vi "PayloadHPLP.vi"(8 "Modulation type LP":enum16{"QPSK(4QAM)", "64QAM", "16QAM", "BPSK"}(ring), 11 "Modulation type HP":enum16{"QPSK(4QAM)", "64QAM", "16QAM", "BPSK"}(ring)) -> (2 "Payload_LP":i32=720, 3 "Payload_HP":i32=720)   [LabVIEW 2022 SP3]
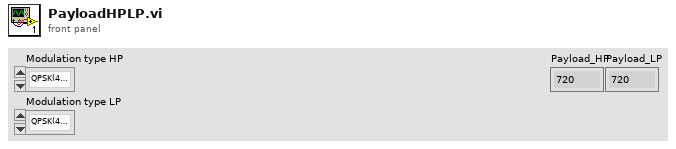
[diagram p1: front panel]
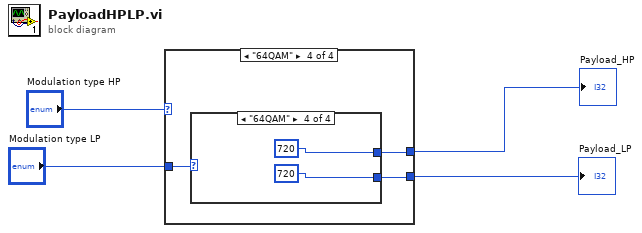
[diagram p0: block diagram]
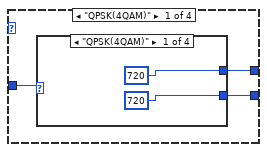
[diagram p2: hidden frame]
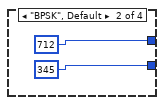
[diagram p3: hidden frame]
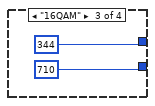
[diagram p4: hidden frame]
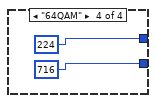
[diagram p5: hidden frame]
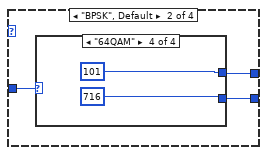
[diagram p6: hidden frame]
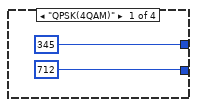
[diagram p7: hidden frame]
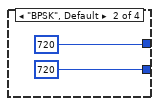
[diagram p8: hidden frame]
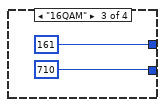
[diagram p9: hidden frame]
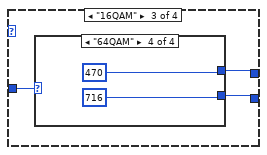
[diagram p10: hidden frame]
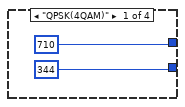
[diagram p11: hidden frame]
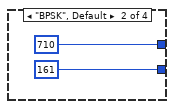
[diagram p12: hidden frame]
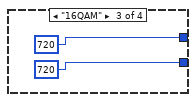
[diagram p13: hidden frame]
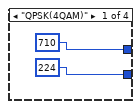
[diagram p14: hidden frame]
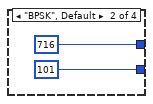
[diagram p15: hidden frame]
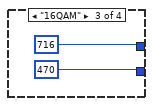
[diagram p16: hidden frame]
diagram:
  n1 = case shown="\"64QAM\"" "Modulation type HP" {
    tunnel: "Modulation type LP" -> [w7 w18 w29 w40]
    tunnel: [w6 w17 w28 w39] -> w2
    tunnel: [w5 w16 w27 w38] -> w1
    frame "QPSK(4QAM)" {
      n2 = case shown="\"QPSK(4QAM)\"" w7 {
        tunnel: [720 712 344 224] -> w6
        tunnel: [720 345 710 716] -> w5
        frame "QPSK(4QAM)" {
        }
        frame "BPSK", Default {
        }
        frame "16QAM" {
        }
        frame "64QAM" {
        }
      }
    }
    frame "BPSK", Default {
      n3 = case shown="\"64QAM\"" w18 {
        tunnel: [345 720 161 101] -> w17
        tunnel: [712 720 710 716] -> w16
        frame "QPSK(4QAM)" {
        }
        frame "BPSK", Default {
        }
        frame "16QAM" {
        }
        frame "64QAM" {
        }
      }
    }
    frame "16QAM" {
      n4 = case shown="\"64QAM\"" w29 {
        tunnel: [710 710 720 470] -> w28
        tunnel: [344 161 720 716] -> w27
        frame "QPSK(4QAM)" {
        }
        frame "BPSK", Default {
        }
        frame "16QAM" {
        }
        frame "64QAM" {
        }
      }
    }
    frame "64QAM" {
      n5 = case shown="\"64QAM\"" w40 {
        tunnel: [710 716 716 720] -> w39
        tunnel: [224 101 470 720] -> w38
        frame "QPSK(4QAM)" {
        }
        frame "BPSK", Default {
        }
        frame "16QAM" {
        }
        frame "64QAM" {
        }
      }
    }
  }
  "Payload_HP" <- w2
  "Payload_LP" <- w1
